vi "CleanUp.vi"(0 "object in":refnum<class "NativeSubTemplate.lvclass">, 5 "Error In":errorcluster) -> (14 "object out":refnum<class "NativeSubTemplate.lvclass">, 19 "Error Out":errorcluster)   [LabVIEW 2020, in "NativeSubTemplate.lvclass"]
uses:
  NativeSubTemplate.lvclass
  NativeBaseTemplate/NativeBaseTemplate.lvclass
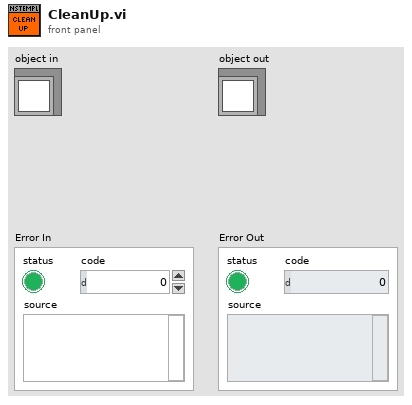
[diagram p1: front panel]
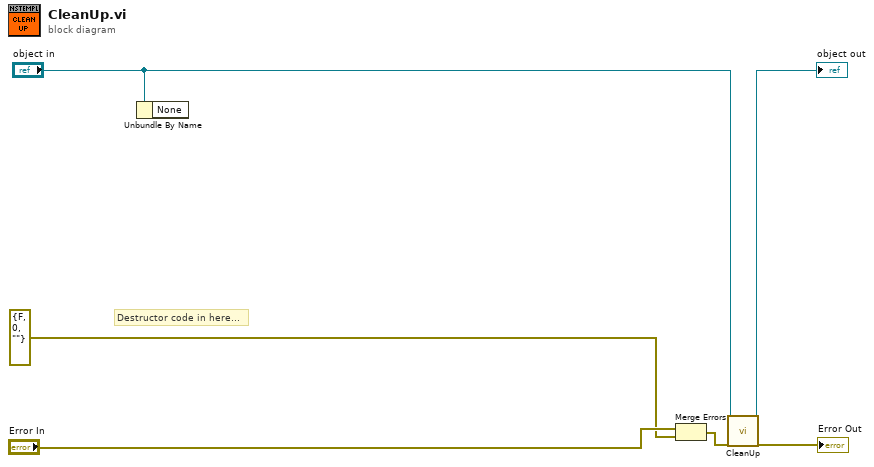
[diagram p0: block diagram]
diagram:
  # "Destructor code in here..."
  n1 = Unbundle By Name("object in") -> ()  [unwired: 1 out]
  n2 = Merge Errors("Error In", errorcluster {"status"=FALSE, "code"=0, "source"=""} ("error in (no error)")) -> (w4:errorcluster)
  n3 = call-parent "CleanUp.vi"("object in"="object in", "Error In"=w4) -> ("object out"=→"object out":refnum<class "NativeSubTemplate.lvclass">, "Error Out"=→"Error Out":errorcluster)  [unwired: 16 in]
